vi "TCP Read Bytes.vi"(8 "error in (no error)":errorcluster, 9 "timeout (1000 ms)":i32=1000, 10 "bytes to read (100)":i32=100, 11 "Connection.TCP":refnum<class "Connection.TCP.lvclass">) -> (0 "error out":errorcluster, 1 "timed out":bool, 2 "Bytes":u8[](array[numeric]) format="%08b", 3 "Connection.TCP":refnum<class "Connection.TCP.lvclass">, 4 "connected":bool)   [LabVIEW 2013, in "Connection.TCP_GOSPL.lvlib" / "Connection.TCP.lvclass"]
uses:
  Connection.TCP.lvclass
  Connection.TCP.lvclass/Connection.TCP.ctl
  Connection/Connection.lvclass
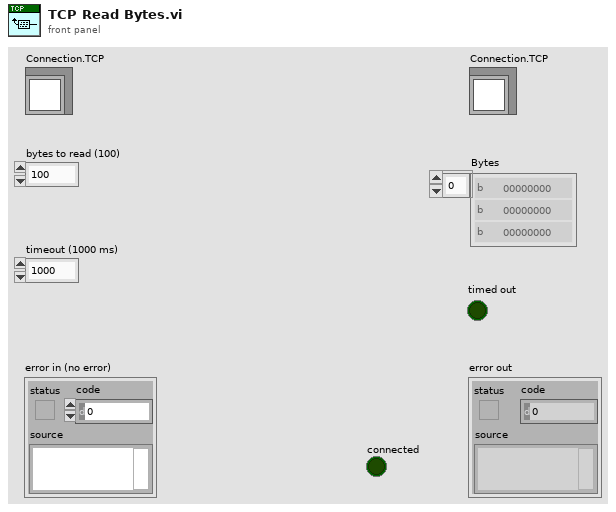
[diagram p1: front panel]
types:
  T1 = enum16{"Standard", "Buffered", "CRLF", "Immediate"}
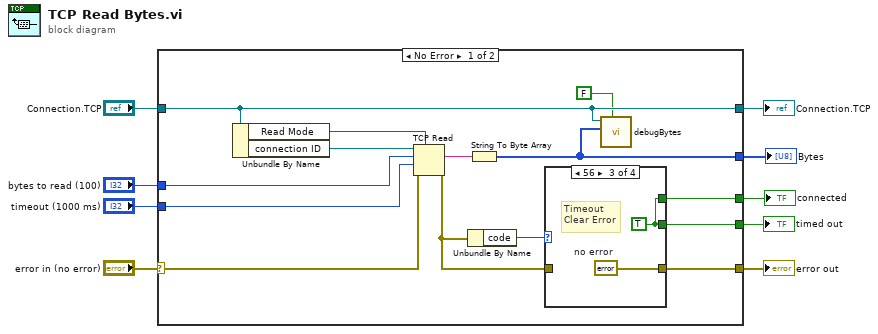
[diagram p0: block diagram]
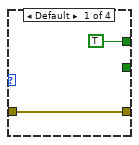
[diagram p2: hidden frame]
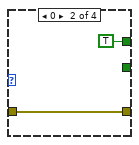
[diagram p3: hidden frame]
diagram:
  n1 = case shown="No Error" "error in (no error)" {
    selector: "error in (no error)" -> [w22 w32]
    tunnel: [w15 w32] -> w8
    tunnel: [w12 w31] -> w6
    tunnel: "Connection.TCP" -> [w12 w31]
    tunnel: [w11 _] -> w5
    tunnel: "bytes to read (100)" -> [w18 _]
    tunnel: "timeout (1000 ms)" -> [w17 _]
    tunnel: [w16 _] -> w2
    tunnel: [w14 _] -> w1
    frame No Error {
      n2 = Unbundle By Name(w12) -> ("Read Mode"=w13:T1, "connection ID"=w23:refnum<k5>)
      n3 = TCP Read(connection ID=w23, bytes to read=w18, error in (no error)=w22, 7:w13, 9:w17) -> (data out=w21:string, error out=w19:errorcluster)  [unwired: 1 out]
      n4 = Unbundle By Name(w19) -> ("code"=w20:i32)
      n5 = String To Byte Array(string=w21) -> (unsigned byte array=w11:u8[])
      n6 = case shown="56" w20 {
        tunnel: [w25 w27 w28 w30] -> w15
        tunnel: w19 -> [w25 w27 _ w30]
        tunnel: [_ _ w29 _] -> w16
        tunnel: [TRUE TRUE w29 _] -> w14
        frame Default {
        }
        frame 0 {
        }
        frame 56 {
          w28 = errorcluster {"status"=FALSE, "code"=0, "source"=""}  # no error
          w29 = TRUE
          # "Timeout\nClear Error"
        }
        frame 66 {
          # "Disconnection\nby peer"
        }
      }
      n7 = call "debugBytes.vi"("outgoing?"=FALSE, "Bytes"=w11, "Connection in"=w12) -> ()  [unwired: 7 in, 2 out]
    }
    frame Error {
    }
  }
  "error out" <- w8
  "Connection.TCP" <- w6
  "Bytes" <- w5
  "timed out" <- w2
  "connected" <- w1
